vi "Supervisor_Set_Mode.vi"(8 "error in (no error)":errorcluster={"status"=FALSE, "code"=0, "source"="\"\""}, 10 "current state":string, 11 "Requested mode":string) -> (0 "error out":errorcluster={"status"=FALSE, "code"=0, "source"="\"\""}, 2 "status ok":bool, 3 "Accepted mode or rejection":string)   [LabVIEW 2026]
doc: "INTENT: Enforce Manual/Auto separation. LOGIC: Change only from stopped/idle safe state with no outstanding leases."
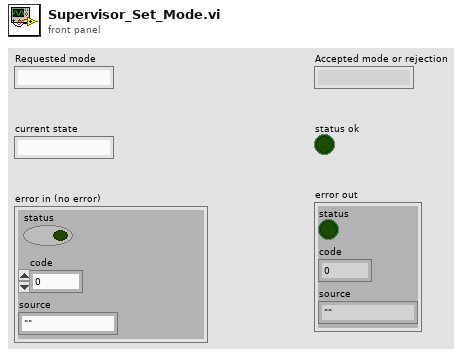
[diagram p1: front panel]
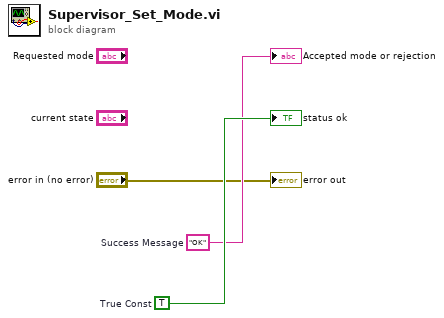
[diagram p0: block diagram]
diagram:
  w3 = TRUE  # True Const
  w2 = "OK"  # Success Message
  "Accepted mode or rejection" <- w2
  "status ok" <- w3
  "error out" <- "error in (no error)"
